vi "Druck_to_Pa.vi"(0 "V_zero":dbl=0.0353, 4 "P_ambient_Pa":dbl=94000.0, 5 "P_FS_gauge_Pa":dbl=1400000.0, 6 "V_FS":dbl=5.0, 7 "V_in":dbl) -> (1 "P_gauge_Pa":dbl, 2 "Out_of_range":bool, 3 "P_abs_Pa":dbl)   [LabVIEW 2025]
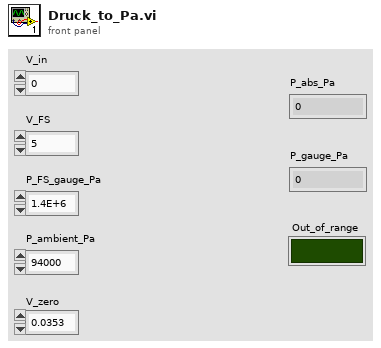
[diagram p1: front panel]
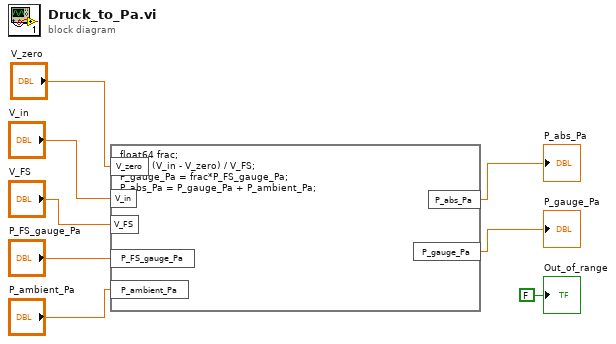
[diagram p0: block diagram]
diagram:
  n1 = formula code="float64 frac;\nfrac = (V_in - V_zero) / V_FS;\nP_gauge_Pa = frac*P_FS_gauge_Pa;\nP_abs_Pa = P_gauge_Pa + P_ambient_Pa;"("V_in"="V_in", "V_FS"="V_FS", "P_FS_gauge_Pa"="P_FS_gauge_Pa", "P_ambient_Pa"="P_ambient_Pa", "V_zero"="V_zero") -> ("P_abs_Pa"=→"P_abs_Pa":dbl, "P_gauge_Pa"=→"P_gauge_Pa":dbl)
  "Out_of_range" <- FALSE ("Out_of_range")
